vi "[ce] CalcExpress - Abort Evaluation.vi"(6 "error in":errorcluster, 9 "CE InstanceRef":T1) -> (0 "error out":errorcluster, 3 "dup CE InstanceRef":T1)   [LabVIEW 2021]
doc: "This VI aborts evaluation of a CalcExpress script associated with <b>CE InstanceRef</b>. Refer to the VI help for more details.\n\n::: CalcExpress Toolkit :::\nCopyright (c) 2000-2026 Konstantin Shifershteyn. All rights reserved."
uses:
  cetypes.llb/CalcExpress Instance RefNum.ctl
  cersrc/celveng32.dll
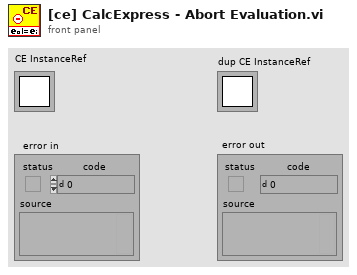
[diagram p1: front panel]
types:
  T1 = typedef "CalcExpress Instance RefNum.ctl" = refnum<k1>
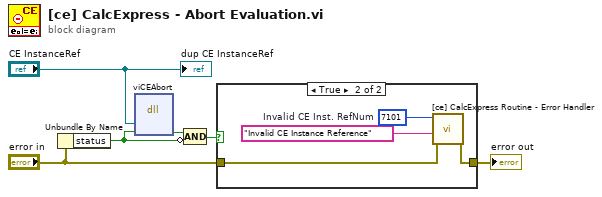
[diagram p0: block diagram]
diagram:
  n1 = Unbundle By Name("error in") -> ("status"=w2:bool)
  n2 = dll-call lib="C:/LV Projects/CalcExpress 40 LV2021/vi.lib/addons/CalcExpress/cersrc/celveng*.dll" fn="viCEAbort"("iRef"="CE InstanceRef", "erf"=w2) -> ("erf"=w3:bool)  [unwired: 5 in, 2 out]
  n3 = Compound Arithmetic op=AND(w3, invert w2) -> (w6:bool)
  n4 = case shown="True" w6 {
    tunnel: "error in" -> [w7 w9]
    tunnel: [w7 w11] -> w4
    frame False {
    }
    frame True {
      w8 = 7101  # Invalid CE Inst. RefNum
      n5 = call "[ce] CalcExpress Routine - Error Handler.vi"("error in"=w9, "error msg"="Invalid CE Instance Reference" ("error description"), "error code"=w8) -> ("error out"=w11:errorcluster)  [unwired: 6 in]
    }
  }
  "error out" <- w4
  "dup CE InstanceRef" <- "CE InstanceRef"
